vi "Set Logger Enqueuer.vi"(8 "error in":errorcluster, 10 "Logger":refnum<class "Message Enqueuer.lvclass">, 11 "Project Manager in":refnum<class "Project Manager.lvclass">) -> (0 "error out":errorcluster, 3 "Project Manager out":refnum<class "Project Manager.lvclass">)   [LabVIEW 2026, in "Project Manager.lvclass"]
doc: "Set the logger enqueuer for a Logger Client."
uses:
  Project Manager.lvclass
  <vilib>/ActorFramework/Message Enqueuer/Message Enqueuer.lvclass
  Project Manager.lvclass/Project Manager.ctl
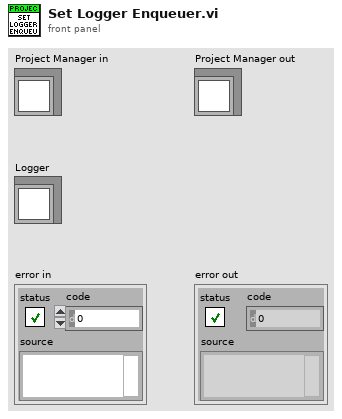
[diagram p1: front panel]
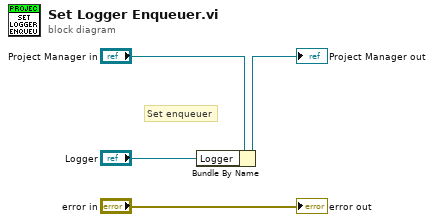
[diagram p0: block diagram]
diagram:
  # "Set enqueuer"
  n1 = Bundle By Name(cluster="Project Manager in", "Logger"="Logger") -> (→"Project Manager out":refnum<class "Project Manager.lvclass">)
  "error out" <- "error in"
